vi "MQTT Client - Connect.vi"(0 "MQTT Session":T3, 7 "Clean Start":bool=TRUE, 11 "error in (no error)":errorcluster, 12 "Connect Properties (v5)":T2[](array[typedef]) {"Property" items=[" Session Expiry Interval           "=17, " Authentication Method             "=21, " Authentication Data               "=22, " Request Problem Information       "=23, " Request Response Information      "=25, " Receive Maximum                   "=33, " Topic Alias Maximum               "=34, " User Property                     "=38, " Maximum Packet Size               "=39]}) -> (4 "MQTT Session out":T3, 6 "Session Present?":bool, 8 "Assigned Client Identifier":string, 14 "Connack Properties (v5)":T1[](array[typedef]) {"Property" items=[" Session Expiry Interval           "=17, " Assigned Client Identifier        "=18, " Server Keep Alive                 "=19, " Authentication Method             "=21, " Authentication Data               "=22, " Response Information              "=26, " Server Reference                  "=28, " Reason String                     "=31, " Receive Maximum                   "=33, " Topic Alias Maximum               "=34, " Maximum QoS                       "=36, " Retain Available                  "=37, " User Property                     "=38, " Maximum Packet Size               "=39, " Wildcard Subscription Available   "=40, " Subscription Identifier Available "=41, " Shared Subscription Available     "=42]}, 15 "error out":errorcluster)   [LabVIEW 2019, in "KoRE-MQTT.lvlib"]
doc: "<b>Description:</b> This VI establishes a connection to an MQTT broker using the specified session parameters and properties. It handles the connection process, including client identification and optional MQTT v5 properties if applicable.\n\n<b>Input Terminals:</b>\n- <b>MQTT Session [0]</b>: Reference to the MQTT session to be connected.\n- <b>Clean Start? [7]</b>: Boolean value indicating whether to initiate a clean session on the broker.\n- <b>Assigned Client Identifier [11]</b>: Unique identifier for the MQTT client used during the connection process.\n- <b>Connect Properties (v5) [12]</b>: Optional array of Property and Value pairs specifically applicable for MQTT v5 connections, allowing additional connection properties.\n\n<b>Output Terminals:</b>\n- <b>MQTT Session out [4]</b>: Reference to the established MQTT session after the connection has been made.\n- <b>Session Present? [6]</b>: Boolean output indicating whether the session was previously present, relevant for clean sessions.\n- <b>Connack Properties (v5) [15]</b>: Optional array of Property and Value pairs returned by the MQTT Broker in MQTT v5, providing connection acknowledgment properties.\n\n\n<b>Input Terminals:</b>\n- <b>MQTT session [0]</b>: Reference to the active MQTT session that needs to be closed.\n\nCopyright (c) 2025 KoRElibs.com\nSPDX-License-Identifier: EUPL-1.2\n\nThis VI is licensed under the European Union Public License (EUPL) Version 1.2. You may use this VI unmodified in proprietary works. If you distribute a modified version of this file, the modified file must be released under the EUPL-1.2. Full license: https://joinup.ec.europa.eu/asset/eupl/eupl/1.2/"
uses:
  KoRE-MQTT.lvlib
  TypeDefs/MQTT Client Session.ctl
  TypeDefs/MQTT Property - CONNECT.ctl
  TypeDefs/MQTT Property - CONNACK.ctl
  TypeDefs/MQTT Version.ctl
  Private/TypeDefs/MQTT Packet - Type.ctl
  Private/MQTT Session - Reset Keep Alive Timer.vi
  Private/MQTT Data Stream - Write Packet.vi
  Private/MQTT Data - Encode Varint.vi
panel:
  in  "Keep Alive":u16
  out "CONNACK":string
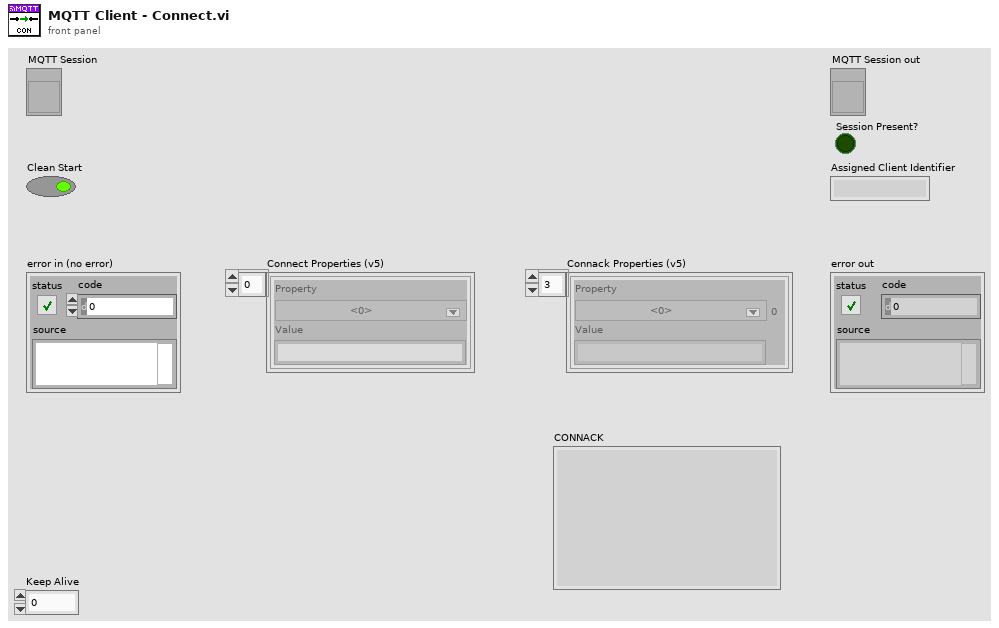
[diagram p1: front panel]
types:
  T1 = typedef "KoRE-MQTT.lvlib/MQTT Property - CONNACK.ctl" = cluster{"Property":u8, "Value":string}
  T2 = typedef "KoRE-MQTT.lvlib/MQTT Property - CONNECT.ctl" = cluster{"Property":u8, "Value":string}
  T3 = typedef "KoRE-MQTT.lvlib/MQTT Client Session.ctl" = refnum<vi>
  T4 = typedef "KoRE-MQTT.lvlib/MQTT Client Session - Data.ctl" = cluster{"TCP ref":refnum<k5>, "Next Packet Id":u16, "Version":u8, "Host":string, "Port":u16, "Ping Delta":u32, "Username":string, "Password":string, "Will QoS":u8, "Will Retain":bool, "Will Topic":string, "Will Payload":string, "TCP Timeout":i32, "Semaphore":T5, "In-Flight Messages":variant, "Close":bool, "Last Send":u32, "Keep Alive":u16, "Last Ping RTT":u32, "Last Ping":u32, "Will Properties":T6[], "Session Expiry Interval":u32, "Maximum QoS":u8, "Retain Available":bool, "Server Maximum Packet Size":u32, "Client Identifier":string, "Server Topic Alias Maximum":u16, "Wildcard Subscription Available":bool, "Subscription Identifier Available":bool, "Shared Subscription Available":bool, "Connect Properties":T2[], "Client Maximum Packet Size":u32, "Client Topic Alias Maximum":u16, "Server Receive Maximum":u16, "Client Receive Maximum":u16, "TLS cfg":refnum<k36>, "Subscriptions":T7[]}
  T5 = typedef "Semaphore RefNum" = refnum<k1>
  T6 = typedef "KoRE-MQTT.lvlib/MQTT Property - Will.ctl" = cluster{"Property":u8, "Value":string}
  T7 = typedef "KoRE-MQTT.lvlib/MQTT Subscription - Info.ctl" = cluster{"Packet Id":u16, "Index":u16, "Identifier":u32, "QoS":u8, "Topic Filter":string, "Reason Code":u8, "Reason String":string, "Granted":bool}
  T8 = typedef "KoRE-MQTT.lvlib/MQTT Packet - Type.ctl" = enum32{"Reserved", "CONNECT", "CONNACK", "PUBLISH", "PUBACK", "PUBREC", "PUBREL", "PUBCOMP", "SUBSCRIBE", "SUBACK", "UNSUBSCRIBE", "UNSUBACK", "PINGREQ", "PINGRESP", "DISCONNECT", "AUTH"}
  T9 = typedef "KoRE-MQTT.lvlib/MQTT Version.ctl" = u16
  T10 = typedef "KoRE-MQTT.lvlib/MQTT Packet - Fixed Header.ctl" = cluster{"MessageType":T8, "DUP Flag":bool, "QoS Level":u8, "RETAIN":bool, "Remaining Length":u32}
  T11 = typedef "KoRE-MQTT.lvlib/MQTT Property - GENERIC.ctl" = cluster{"Property":T12, "Value":string}
  T12 = typedef "KoRE-MQTT.lvlib/MQTT Property Type.ctl" = u8
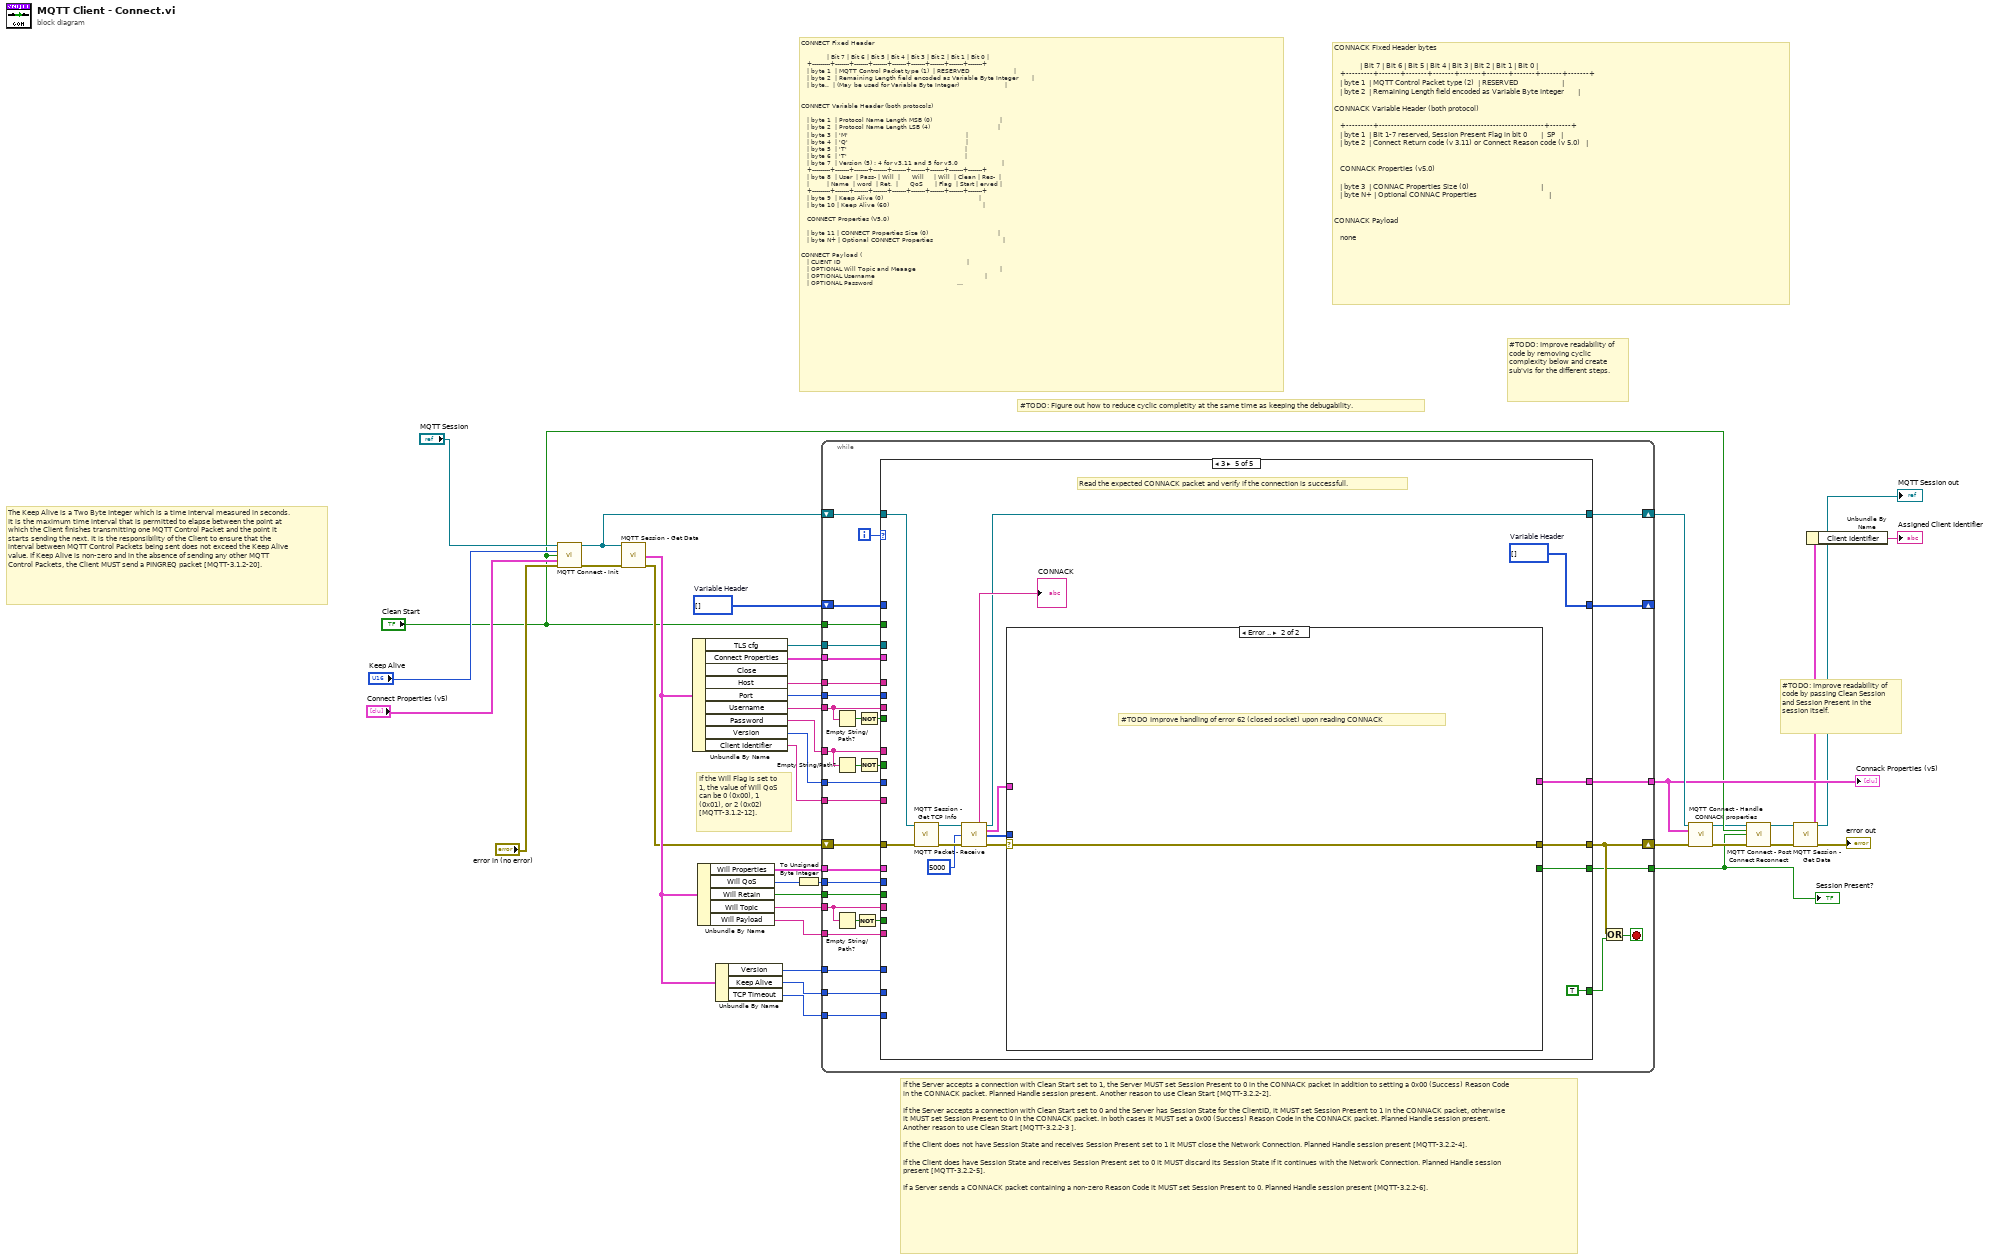
[diagram p0: block diagram]
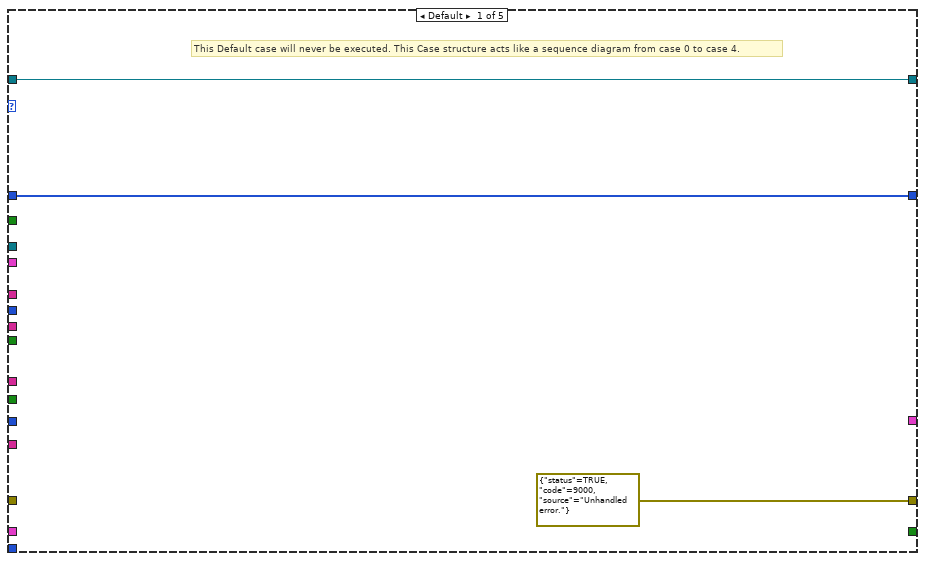
[diagram p2: hidden frame]
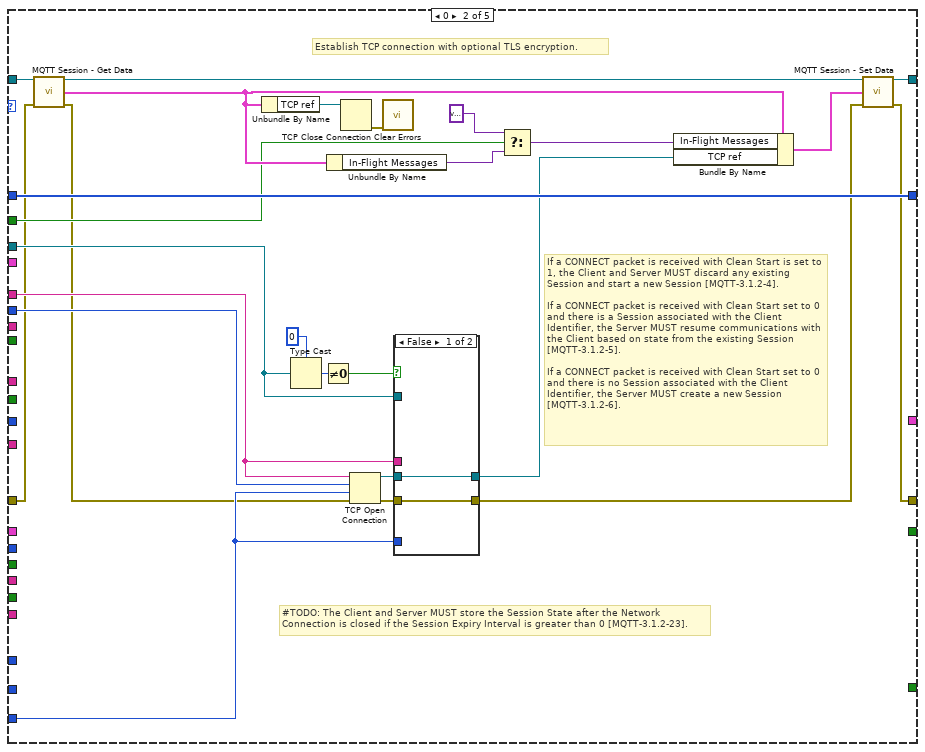
[diagram p3: hidden frame]
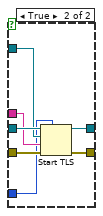
[diagram p4: hidden frame]
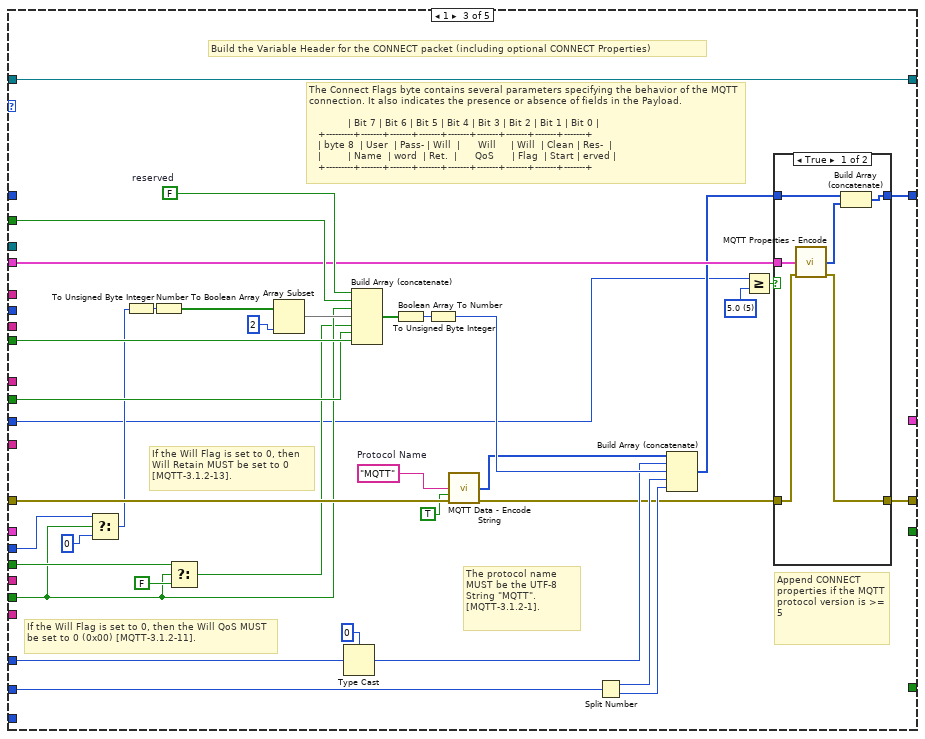
[diagram p5: hidden frame]
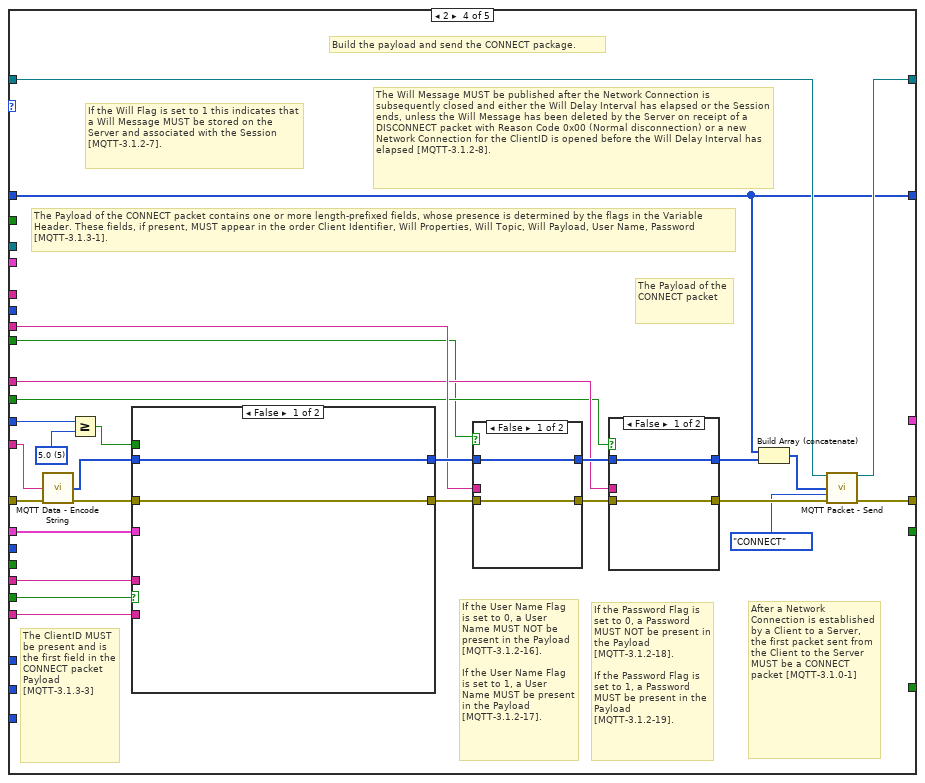
[diagram p7: hidden frame]
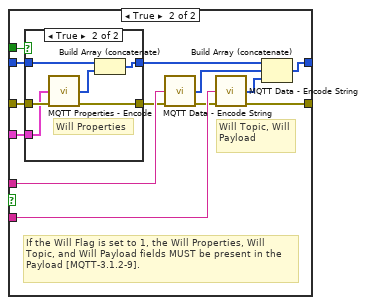
[diagram p8: hidden frame]
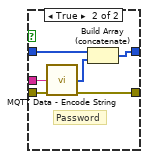
[diagram p10: hidden frame]
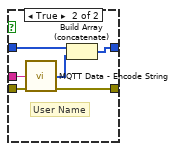
[diagram p11: hidden frame]
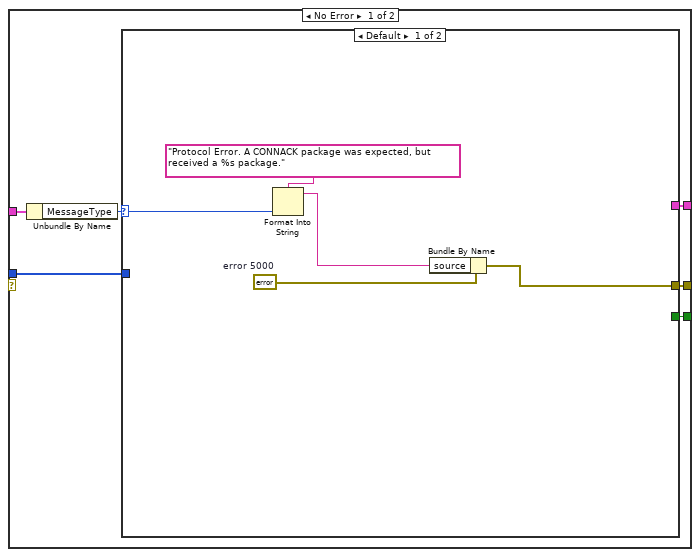
[diagram p12: hidden frame]
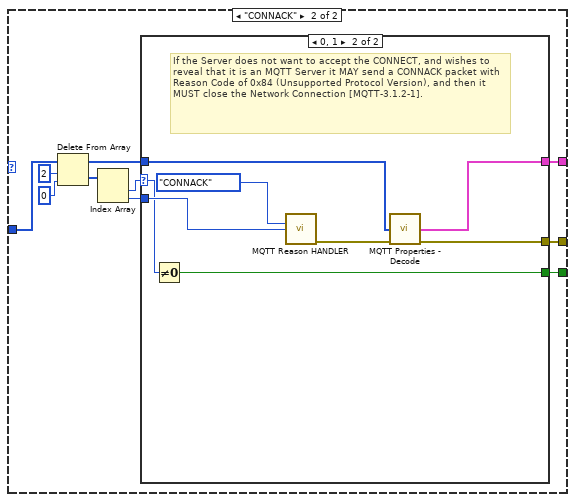
[diagram p13: hidden frame]
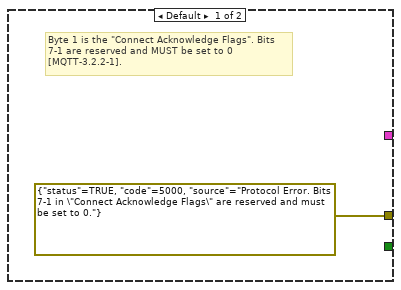
[diagram p14: hidden frame]
diagram:
  w34 = u8[] []  # Variable Header
  # "#TODO: Improve readability of code by removing cyclic complexity below and create sub'vis for the different steps."
  # "#TODO: Improve readability of code by passing Clean Session and Session Present in the session itself."
  # "#TODO: Figure out how to reduce cyclic completity at the same time as keeping the debugability."
  # "If the Server accepts a connection with Clean Start set to 1, the Server MUST set Session Present to 0 in the CONNACK packet in addition to setting a 0x00 (Success) Reason Code in the CONNACK packet.\tPlanned\tHandle session present. Another reason to use Clean Start [MQTT-3.2.2-2].\n\nIf the Server accepts a connection with Clean Start set to 0 and the Server has Session State for the ClientID, it MUST set Session Present to 1 in the CONNACK packet, otherwise it MUST set Session Present to 0 in the CONNACK packet. In both cases it MUST set a 0x00 (Success) Reason Code in the CONNACK packet.\tPlanned\tHandle session present. Another reason to use Clean Start [MQTT-3.2.2-3\t].\n\nIf the Client does not have Session State and receives Session Present set to 1 it MUST close the Network Connection.\tPlanned\tHandle session present [MQTT-3.2.2-4].\n\nIf the Client does have Session State and receives Session Present set to 0 it MUST discard its Session State if it continues with the Network Connection.\tPlanned\tHandle session present [MQTT-3.2.2-5].\n\nIf a Server sends a CONNACK packet containing a non-zero Reason Code it MUST set Session Present to 0.\tPlanned\tHandle session present [MQTT-3.2.2-6]."
  # "The Keep Alive is a Two Byte Integer which is a time interval measured in seconds. It is the maximum time interval that is permitted to elapse between the point at which the Client finishes transmitting one MQTT Control Packet and the point it starts sending the next. It is the responsibility of the Client to ensure that the interval between MQTT Control Packets being sent does not exceed the Keep Alive value. If Keep Alive is non-zero and in the absence of sending any other MQTT Control Packets, the Client MUST send a PINGREQ packet [MQTT-3.1.2-20]."
  # "If the Will Flag is set to 1, the value of Will QoS can be 0 (0x00), 1 (0x01), or 2 (0x02) [MQTT-3.1.2-12]."
  # "CONNACK Fixed Header bytes\n\n             | Bit 7 | Bit 6 | Bit 5 | Bit 4 | Bit 3 | Bit 2 | Bit 1 | Bit 0 |\n   +---------+-------+-------+-------+-------+-------+-------+-------+-------+\n   | byte 1  | MQTT Control Packet type (2)  | RESERVED                      |\n   | byte 2  | Remaining Length field encoded as Variable Byte Integer       |\n\nCONNACK Variable Header (both protocol)\n\n   +---------+-------------------------------------------------------+-------+\n   | byte 1  | Bit 1-7 reserved, Session Present Flag in bit 0       |  SP   |\n   | byte 2  | Connect Return code (v 3.11) or Connect Reason code (v 5.0)   |\n\n\n   CONNACK Properties (v5.0)\n\n   | byte 3  | CONNAC Properties Size (0)                                    |\n   | byte N+ | Optional CONNAC Properties                                    |\n\n\nCONNACK Payload\n\n   none"
  # "CONNECT Fixed Header\n\n             | Bit 7 | Bit 6 | Bit 5 | Bit 4 | Bit 3 | Bit 2 | Bit 1 | Bit 0 |\n   +---------+-------+-------+-------+-------+-------+-------+-------+-------+\n   | byte 1  | MQTT Control Packet type (1)  | RESERVED                      |\n   | byte 2  | Remaining Length field encoded as Variable Byte Integer       |\n   | byte..  | (May be used for Variable Byte Integer)                       | \n\n\nCONNECT Variable Header (both protocols)\n\n   | byte 1  | Protocol Name Length MSB (0)                                  | \n   | byte 2  | Protocol Name Length LSB (4)                                  |\n   | byte 3  | 'M'                                                           |\n   | byte 4  | 'Q'                                                           |\n   | byte 5  | 'T'                                                           |\n   | byte 6  | 'T'                                                           |\n   | byte 7  | Version (5) : 4 for v3.11 and 5 for v5.0                      |\n   +---------+-------+-------+-------+-------+-------+-------+-------+-------+\n   | byte 8  | User  | Pass- | Will  |      Will     | Will  | Clean | Res-  |\n   |         | Name  | word  | Ret.  |      QoS      | Flag  | Start | erved |\n   +---------+-------+-------+-------+-------+-------+-------+-------+-------+\n   | byte 9  | Keep Alive (0)                                                | \n   | byte 10 | Keep Alive (60)                                               |\n\n   CONNECT Properties (V5.0)\n\n   | byte 11 | CONNECT Properties Size (0)                                   |\n   | byte N+ | Optional CONNECT Properties                                   |\n\nCONNECT Payload (\n   | CLIENT ID                                                               |\n   | OPTIONAL Will Topic and Meaage                                          |\n   | OPTIONAL Username                                                       |\n   | OPTIONAL Password                                                      |"
  n1 = call "MQTT Connect - Init.vi"("MQTT ref in"="MQTT Session", "Keep Alive"="Keep Alive", "Clean start"="Clean Start", "Connect Properties"="Connect Properties (v5)", "error in (no error)"="error in (no error)") -> ("MQTT ref out"=w19:T3, "error out"=w9:errorcluster)  [unwired: 9 in]
  n2 = call "MQTT Session - Get Data.vi"("mqtt ref in"=w19, "error in"=w9) -> ("mqtt ref data"=w18:T4, "error out"=w8:errorcluster)  [unwired: 11 in, 1 out]
  n3 = Unbundle By Name(w18) -> ("TLS cfg"=w15:refnum<k36>, "Connect Properties"=w35:T2[], "Host"=w39:string, "Port"=w38:u16, "Username"=w37:string, "Password"=w36:string, "Version"=w10:u8, "Client Identifier"=w11:string)  [unwired: 1 out]
  n4 = Unbundle By Name(w18) -> ("Will Properties"=w24:T6[], "Will QoS"=w30:u8, "Will Retain"=w31:bool, "Will Topic"=w32:string, "Will Payload"=w33:string)
  n5 = Unbundle By Name(w18) -> ("Version"=w27:u8, "Keep Alive"=w28:u16, "TCP Timeout"=w29:i32)
  n6 = To Unsigned Byte Integer(number=w30) -> (unsigned 8bit integer=w26:u8)
  n7 = while {
    shift-right: [w50] -> w16
    shift-left: w8 -> [w72]
    tunnel: w11 -> [w71]
    shift-right: [w70] -> _
    shift-left: w34 -> [w69]
    tunnel: w39 -> [w66]
    tunnel: w38 -> [w65]
    tunnel: w32 -> [w64]
    tunnel: w37 -> [w63]
    tunnel: w36 -> [w62]
    tunnel: w33 -> [w61]
    tunnel: w28 -> [w57]
    tunnel: w26 -> [w53]
    tunnel: w31 -> [w52]
    tunnel: "Clean Start" -> [w51]
    tunnel: w27 -> [w49]
    tunnel: w35 -> [w48]
    tunnel: w29 -> [w47]
    shift-right: [w45] -> w23
    shift-left: w19 -> [w46]
    tunnel: w24 -> [w44]
    tunnel: [w43] -> w17
    tunnel: w15 -> [w42]
    tunnel: w10 -> [w41]
    tunnel: [w40] -> w6
    i -> [w73]
    stop <- w68 stop-if-true
    n8 = Empty String/Path?(string/path=w63) -> (empty?=w59:bool)
    n9 = Empty String/Path?(string/path=w62) -> (empty?=w60:bool)
    n10 = Empty String/Path?(string/path=w64) -> (empty?=w58:bool)
    n11 = Not(x=w58) -> (.not. x?=w56:bool)
    n12 = Not(x=w59) -> (.not. x?=w54:bool)
    n13 = Not(x=w60) -> (.not. x?=w55:bool)
    n14 = case shown="3" w73 {
      tunnel: w72 -> [_ w80 w146 w179 w230]
      tunnel: [errorcluster {"status"=TRUE, "code"=9000, "source"="Unhandled error."} w77 w115 w163 w225] -> w50
      tunnel: w71 -> [_ _ _ w166 _]
      tunnel: [w76 w102 w113 w159 w236] -> w70
      tunnel: w69 -> [w76 w102 _ w159 _]
      tunnel: [_ _ _ _ TRUE] -> w67
      tunnel: w66 -> [_ w86 _ _ _]
      tunnel: w65 -> [_ w101 _ _ _]
      tunnel: w64 -> [_ _ _ w178 _]
      tunnel: w63 -> [_ _ _ w176 _]
      tunnel: w62 -> [_ _ _ w175 _]
      tunnel: w61 -> [_ _ _ w177 _]
      tunnel: w55 -> [_ _ w134 w174 _]
      tunnel: w54 -> [_ _ w135 w173 _]
      tunnel: w56 -> [_ _ w122 w169 _]
      tunnel: w57 -> [_ _ w123 _ _]
      tunnel: w53 -> [_ _ w130 _ _]
      tunnel: w52 -> [_ _ w127 _ _]
      tunnel: w51 -> [_ w93 w133 _ _]
      tunnel: w49 -> [_ _ w125 _ _]
      tunnel: w48 -> [_ _ w117 _ _]
      tunnel: w47 -> [_ w85 _ _ _]
      tunnel: w46 -> [w74 w100 w131 w161 w227]
      tunnel: [w74 w97 w131 w160 w224] -> w45
      tunnel: w44 -> [_ _ _ w170 _]
      tunnel: [_ _ _ _ w231] -> w43
      tunnel: w42 -> [_ w84 _ _ _]
      tunnel: w41 -> [_ _ w112 w165 _]
      tunnel: [_ _ _ _ w226] -> w40
      frame Default {
        # "This Default case will never be executed. This Case structure acts like a sequence diagram from case 0 to case 4."
      }
      frame 0 {
        # "Establish TCP connection with optional TLS encryption."
        # "#TODO: The Client and Server MUST store the Session State after the Network Connection is closed if the Session Expiry Interval is greater than 0 [MQTT-3.1.2-23]."
        # "If a CONNECT packet is received with Clean Start is set to 1, the Client and Server MUST discard any existing Session and start a new Session [MQTT-3.1.2-4].\n\nIf a CONNECT packet is received with Clean Start set to 0 and there is a Session associated with the Client Identifier, the Server MUST resume communications with the Client based on state from the existing Session [MQTT-3.1.2-5]. \n\nIf a CONNECT packet is received with Clean Start set to 0 and there is no Session associated with the Client Identifier, the Server MUST create a new Session [MQTT-3.1.2-6]."
        n15 = call "MQTT Session - Get Data.vi"("mqtt ref in"=w100, "error in"=w80) -> ("mqtt ref out"=w98:T3, "mqtt ref data"=w94:T4, "error out"=w79:errorcluster)  [unwired: 11 in]
        n16 = Unbundle By Name(w94) -> ("TCP ref"=w96:refnum<k5>)
        n17 = Type Cast(type=u64 0, x=w84) -> (*(type *) &x=w82:u64)
        n18 = Not Equal To 0?(x=w82) -> (x != 0?=w81:bool)
        n19 = Unbundle By Name(w94) -> ("In-Flight Messages"=w92:variant)
        n20 = TCP Close Connection(connection ID=w96) -> (error out=w95:errorcluster)  [unwired: 2 in, 1 out]
        n21 = TCP Open Connection(address=w86, remote port or service name=w101, timeout ms (60000)=w85, error in (no error)=w79) -> (connection ID=w89:refnum<k5>, error out=w87:errorcluster)  [unwired: 1 in]
        n22 = call <vilib>:"Clear Errors.vi"("error in (no error)"=w95) -> ()  [unwired: 5 in, 2 out]
        n23 = case shown="False" w81 {
          tunnel: w89 -> [w104 w111]
          tunnel: [w104 w110] -> w88
          tunnel: w87 -> [w103 w109]
          tunnel: [w103 w108] -> w78
          tunnel: w84 -> [_ w107]
          tunnel: w86 -> [_ w106]
          tunnel: w85 -> [_ w105]
          frame False {
          }
          frame True {
            n24 = Start TLS(7:w105, 8:w109, 9:w106, 10:w107, 11:w111) -> (0:w108:errorcluster, 3:w110:refnum<k5>)  [unwired: 1 in, 1 out]
          }
        }
        n25 = Select(t=variant, s=w93, f=w92) -> (s? t:f=w90:variant)
        n26 = Bundle By Name(cluster=w94, "In-Flight Messages"=w90, "TCP ref"=w88) -> (w99:T4)
        n27 = call "MQTT Session - Set Data.vi"("mqtt ref in"=w98, "mqtt ref data"=w99, "error in"=w78) -> ("mqtt ref out"=w97:T3, "error out"=w77:errorcluster)  [unwired: 11 in]
      }
      frame 1 {
        w119 = T9 5 items=["3.11"=4, "5.0"=5] ("y")
        w136 = FALSE  # reserved
        w138 = "MQTT"  # Protocol Name
        # "Append CONNECT properties if the MQTT protocol version is >= 5"
        # "If the Will Flag is set to 0, then Will Retain MUST be set to 0 [MQTT-3.1.2-13]."
        # "If the Will Flag is set to 0, then the Will QoS MUST be set to 0 (0x00) [MQTT-3.1.2-11]."
        # "Build the Variable Header for the CONNECT packet (including optional CONNECT Properties)"
        # "The Connect Flags byte contains several parameters specifying the behavior of the MQTT connection. It also indicates the presence or absence of fields in the Payload.   \n\n             | Bit 7 | Bit 6 | Bit 5 | Bit 4 | Bit 3 | Bit 2 | Bit 1 | Bit 0 |\n   +---------+-------+-------+-------+-------+-------+-------+-------+-------+\n   | byte 8  | User  | Pass- | Will  |      Will     | Will  | Clean | Res-  |\n   |         | Name  | word  | Ret.  |      QoS      | Flag  | Start | erved |\n   +---------+-------+-------+-------+-------+-------+-------+-------+-------+"
        # "The protocol name MUST be the UTF-8 String \"MQTT\". [MQTT-3.1.2-1]."
        n28 = Select(t=w130, s=w122, f=u8 0) -> (s? t:f=w128:u8)
        n29 = To Unsigned Byte Integer(number=w128) -> (unsigned 8bit integer=w140:u8)
        n30 = Number To Boolean Array(number=w140) -> (Boolean array=w141:bool[])
        n31 = Select(t=w127, s=w122, f=FALSE) -> (s? t:f=w121:bool)
        n32 = Array Subset(array=w141, length=2) -> (w143:bool[])  [unwired: 1 in]
        n33 = Type Cast(type=u8 0, x=w125) -> (*(type *) &x=w124:u8)
        n34 = Build Array (concatenate)(w136, w133, w122, w143, w121, w134, w135) -> (w144:bool[])
        n35 = Boolean Array To Number(Boolean array=w144) -> (number=w145:u32)
        n36 = To Unsigned Byte Integer(number=w145) -> (unsigned 8bit integer=w139:u8)
        n37 = call "MQTT Data - Encode String.vi"("String in"=w138, "To UTF-8?"=TRUE, "error in (no error)"=w146) -> ("Bytes out"=w137:u8[], "error out"=w116:errorcluster)  [unwired: 11 in]
        n38 = Split Number(x=w123) -> (hi(x)=w148:u8, lo(x)=w147:u8)
        n39 = Build Array (concatenate)(w137, w124, w139, w148, w147) -> (w114:u8[])
        n40 = Greater Or Equal?(x=w112, y=w119) -> (x >= y?=w118:bool)
        n41 = case shown="True" w118 {
          tunnel: [w154 w156] -> w113
          tunnel: w117 -> [w153 _]
          tunnel: [w151 w155] -> w115
          tunnel: w116 -> [w150 w155]
          tunnel: w114 -> [w149 w156]
          frame True {
            n42 = call "MQTT Properties - Encode.vi"("MQTT Properties"=w153, "error in (no error)"=w150) -> ("Encoded MQTT Properties"=w152:u8[], "error out"=w151:errorcluster)  [unwired: 12 in]
            n43 = Build Array (concatenate)(w149, w152) -> (w154:u8[])
          }
          frame False {
          }
        }
      }
      frame 2 {
        w168 = T9 5 items=["3.11"=4, "5.0"=5] ("y")
        # "Build the payload and send the CONNECT package."
        # "After a Network Connection is established by a Client to a Server, the first packet sent from the Client to the Server MUST be a CONNECT packet [MQTT-3.1.0-1]"
        # "The ClientID MUST be present and is the first field in the CONNECT packet Payload [MQTT-3.1.3-3]"
        # "The Payload of the CONNECT packet"
        # "The Payload of the CONNECT packet contains one or more length-prefixed fields, whose presence is determined by the flags in the Variable Header. These fields, if present, MUST appear in the order Client Identifier, Will Properties, Will Topic, Will Payload, User Name, Password [MQTT-3.1.3-1]."
        # "If the Password Flag is set to 0, a Password MUST NOT be present in the Payload [MQTT-3.1.2-18]. \n\nIf the Password Flag is set to 1, a Password MUST be present in the Payload [MQTT-3.1.2-19]."
        # "If the User Name Flag is set to 0, a User Name MUST NOT be present in the Payload [MQTT-3.1.2-16].\n\nIf the User Name Flag is set to 1, a User Name MUST be present in the Payload [MQTT-3.1.2-17]."
        # "The Will Message MUST be published after the Network Connection is subsequently closed and either the Will Delay Interval has elapsed or the Session ends, unless the Will Message has been deleted by the Server on receipt of a DISCONNECT packet with Reason Code 0x00 (Normal disconnection) or a new Network Connection for the ClientID is opened before the Will Delay Interval has elapsed [MQTT-3.1.2-8]."
        # "If the Will Flag is set to 1 this indicates that a Will Message MUST be stored on the Server and associated with the Session [MQTT-3.1.2-7]."
        n44 = call "MQTT Data - Encode String.vi"("String in"=w166, "error in (no error)"=w179) -> ("Bytes out"=w171:u8[], "error out"=w172:errorcluster)  [unwired: 12 in]
        n45 = Greater Or Equal?(x=w165, y=w168) -> (x >= y?=w167:bool)
        n46 = case shown="False" w169 {
          tunnel: [w185 w198] -> w183
          tunnel: [w184 w197] -> w180
          tunnel: w178 -> [_ w196]
          tunnel: w177 -> [_ w195]
          tunnel: w172 -> [w185 w194]
          tunnel: w171 -> [w184 w191]
          tunnel: w170 -> [_ w190]
          tunnel: w167 -> [_ w186]
          frame False {
          }
          frame True {
            # "If the Will Flag is set to 1, the Will Properties, Will Topic, and Will Payload fields MUST be present in the Payload [MQTT-3.1.2-9]."
            # "Will Topic, Will Payload"
            n47 = case shown="True" w186 {
              tunnel: w194 -> [w199 w206]
              tunnel: [w199 w205] -> w193
              tunnel: [w200 w204] -> w192
              tunnel: w191 -> [w200 w203]
              tunnel: w190 -> [_ w202]
              frame False {
              }
              frame True {
                # "Will Properties"
                n48 = call "MQTT Properties - Encode.vi"("MQTT Properties"=w202, "error in (no error)"=w206) -> ("Encoded MQTT Properties"=w201:u8[], "error out"=w205:errorcluster)  [unwired: 12 in]
                n49 = Build Array (concatenate)(w203, w201) -> (w204:u8[])
              }
            }
            n50 = call "MQTT Data - Encode String.vi"("String in"=w196, "error in (no error)"=w193) -> ("Bytes out"=w188:u8[], "error out"=w189:errorcluster)  [unwired: 12 in]
            n51 = call "MQTT Data - Encode String.vi"("String in"=w195, "error in (no error)"=w189) -> ("Bytes out"=w187:u8[], "error out"=w198:errorcluster)  [unwired: 12 in]
            n52 = Build Array (concatenate)(w192, w188, w187) -> (w197:u8[])
          }
        }
        n53 = case shown="False" w173 {
          tunnel: w180 -> [w216 w222]
          tunnel: [w216 w221] -> w181
          tunnel: [w215 w220] -> w182
          tunnel: w183 -> [w215 w219]
          tunnel: w176 -> [_ w217]
          frame False {
          }
          frame True {
            # "User Name"
            n54 = call "MQTT Data - Encode String.vi"("String in"=w217, "error in (no error)"=w219) -> ("Bytes out"=w218:u8[], "error out"=w220:errorcluster)  [unwired: 12 in]
            n55 = Build Array (concatenate)(w222, w218) -> (w221:u8[])
          }
        }
        n56 = case shown="False" w174 {
          tunnel: w181 -> [w208 w214]
          tunnel: [w208 w213] -> w158
          tunnel: w182 -> [w207 w212]
          tunnel: [w207 w211] -> w164
          tunnel: w175 -> [_ w209]
          frame False {
          }
          frame True {
            # "Password"
            n57 = call "MQTT Data - Encode String.vi"("String in"=w209, "error in (no error)"=w212) -> ("Bytes out"=w210:u8[], "error out"=w211:errorcluster)  [unwired: 12 in]
            n58 = Build Array (concatenate)(w214, w210) -> (w213:u8[])
          }
        }
        n59 = Build Array (concatenate)(w159, w158) -> (w157:u8[])
        n60 = call "MQTT Packet - Send.vi"("mqtt ref in"=w161, "packet data"=w157, "MessageType"=MQTT_Packet_-_Type."CONNECT", "error in (no error)"=w164) -> ("mqtt ref out"=w160:T3, "error out"=w163:errorcluster)  [unwired: 9 in, 1 out]
      }
      frame 3 {
        w236 = u8[] []  # Variable Header
        # "Read the expected CONNACK packet and verify if the connection is successfull."
        n61 = call "MQTT Session - Get TCP Info.vi"("mqtt ref in"=w227, "error in"=w230) -> ("mqtt ref out"=w228:T3, "error out"=w229:errorcluster)  [unwired: 9 in, 3 out]
        n62 = call "MQTT Packet - Receive.vi"("mqtt ref in"=w228, "timeout (global)"=5000, "error in"=w229) -> ("RAW data"=→"CONNACK":string, "mqtt ref out"=w224:T3, "Fixed Header"=w234:T10, "Remaining Data"=w235:u8[], "error out"=w233:errorcluster)  [unwired: 7 in, 1 out]
        n63 = case shown="Error .." w233 {
          selector: w233 -> [_ w268]
          tunnel: w235 -> [w243 _]
          tunnel: [w242 w268] -> w225
          tunnel: w234 -> [w241 _]
          tunnel: [w239 _] -> w231
          tunnel: [w238 _] -> w226
          frame No Error {
            n64 = Unbundle By Name(w241) -> ("MessageType"=w240:T8)
            n65 = case shown="Default" w240 {
              selector: w240 -> [w248 _]
              tunnel: w243 -> [_ w258]
              tunnel: [w247 w257] -> w242
              tunnel: [_ w250] -> w239
              tunnel: [_ w249] -> w238
              frame Default {
                w245 = errorcluster {"status"=TRUE, "code"=5000, "source"=""}  # error 5000
                n66 = Format Into String(format string="Protocol Error. A CONNACK package was expected, but received a %s package." ("source"), w248) -> (resulting string=w244:string)  [unwired: 2 in, 1 out]
                n67 = Bundle By Name(cluster=w245, "source"=w244) -> (w247:errorcluster)
              }
              frame "CONNACK" {
                n68 = Delete From Array(array=w258, length=2, index=0) -> (deleted portion=w252:u8[], array with subset deleted=w251:u8[])
                n69 = Index Array(array=w252) -> (element #1=w255:u8, element #2=w256:u8)  [unwired: 2 in]
                n70 = case shown="0, 1" w255 {
                  selector: w255 -> [_ w261]
                  tunnel: [errorcluster {"status"=TRUE, "code"=5000, "source"="Protocol Error. Bits 7-1 in \"Connect Acknowledge Flags\" are reserved and must be set to 0."} ("error out") w263] -> w257
                  tunnel: w256 -> [_ w266]
                  tunnel: w251 -> [_ w265]
                  tunnel: [_ w262] -> w250
                  tunnel: [_ w260] -> w249
                  frame Default {
                    # "Byte 1 is the \"Connect Acknowledge Flags\". Bits 7-1 are reserved and MUST be set to 0 [MQTT-3.2.2-1]."
                  }
                  frame 0, 1 {
                    # "If the Server does not want to accept the CONNECT, and wishes to reveal that it is an MQTT Server it MAY send a CONNACK packet with Reason Code of 0x84 (Unsupported Protocol Version), and then it MUST close the Network Connection [MQTT-3.1.2-1]."
                    n71 = Not Equal To 0?(x=w261) -> (x != 0?=w260:bool)
                    n72 = call "MQTT Reason HANDLER.vi"("MessageType"=MQTT_Packet_-_Type."CONNACK", "Reason Code"=w266) -> ("error out"=w264:errorcluster)  [unwired: 13 in]
                    n73 = call "MQTT Properties - Decode.vi"("Encoded MQTT Properties"=w265, "error in (no error)"=w264) -> ("MQTT Properties"=w262:T11[], "error out"=w263:errorcluster)  [unwired: 11 in, 1 out]
                  }
                }
              }
            }
          }
          frame Error {
            # "#TODO Improve handling of error 62 (closed socket) upon reading CONNACK"
          }
        }
      }
    }
    n74 = Or(x=w50, y=w67) -> (x .or. y?=w68:bool)
  }
  "Connack Properties (v5)" <- w17
  "Session Present?" <- w6
  n75 = call "MQTT Connect - Handle CONNACK properties.vi"("MQTT session"=w23, "MQTT CONNACK Properties"=w17, "error in (no error)"=w16) -> ("MQTT session out"=w4:T3, "error out"=w7:errorcluster)  [unwired: 11 in]
  n76 = call "MQTT Connect - Post Connect Reconnect.vi"("MQTT Session"=w4, "Clean Start"="Clean Start", "Session present"=w6, "error in"=w7) -> ("MQTT Session out"=w3:T3, "error out"=w2:errorcluster)  [unwired: 10 in]
  n77 = call "MQTT Session - Get Data.vi"("mqtt ref in"=w3, "error in"=w2) -> ("mqtt ref out"=→"MQTT Session out":T3, "mqtt ref data"=w14:T4, "error out"=→"error out":errorcluster)  [unwired: 11 in]
  n78 = Unbundle By Name(w14) -> ("Client Identifier"=→"Assigned Client Identifier":string)
